vi "Sort Frames by Timing.vi"(8 "error in (no error)":errorcluster, 9 "Counter Offset":i32=3, 10 "Max frames per bucket":i32=10, 11 "Outgoing Cyclic Frames":T4[](array[typedef])=[{"Type"=enum."Periodic", "Frame ID"=101, "Payload Length"=8, "VS Offset"=0, "VS Length"=2, "Frame Conversion"="", "Frame.Data"=[0.0, 0.0], "Generation Period"=100, "Time Since Last Generation"=0, "Generation Iterations"=10, "Generation Counter"=0, "Has Protection?"=FALSE, "Protection Configurations"=[], "Has Counter?"=FALSE, "Counter Configurations"=[], "Has Disable?"=FALSE, "Disable VS Index"=0, "Transmit Trigger"=enum."Channel value change", "Trigger VS Index"=0}, {"Type"=enum."Periodic", "Frame ID"=110, "Payload Length"=8, "VS Offset"=2, "VS Length"=2, "Frame Conversion"="", "Frame.Data"=[0.0, 0.0], "Generation Period"=100, "Time Since Last Generation"=0, "Generation Iterations"=10, "Generation Counter"=0, "Has Protection?"=FALSE, "Protection Configurations"=[], "Has Counter?"=FALSE, "Counter Configurations"=[], "Has Disable?"=FALSE, "Disable VS Index"=0, "Transmit Trigger"=enum."Channel value change", "Trigger VS Index"=0}, {"Type"=enum."Periodic", "Frame ID"=1, "Payload Length"=8, "VS Offset"=4, "VS Length"=2, "Frame Conversion"="", "Frame.Data"=[0.0, 0.0], "Generation Period"=10, "Time Since Last Generation"=0, "Generation Iterations"=1, "Generation Counter"=0, "Has Protection?"=FALSE, "Protection Configurations"=[], "Has Counter?"=FALSE, "Counter Configurations"=[], "Has Disable?"=FALSE, "Disable VS Index"=0, "Transmit Trigger"=enum."Channel value change", "Trigger VS Index"=0}, {"Type"=enum."Periodic", "Frame ID"=51, "Payload Length"=8, "VS Offset"=8, "VS Length"=2, "Frame Conversion"="", "Frame.Data"=[0.0, 0.0], "Generation Period"=50, "Time Since Last Generation"=0, "Generation Iterations"=5, "Generation Counter"=0, "Has Protection?"=FALSE, "Protection Configurations"=[], "Has Counter?"=FALSE, "Counter Configurations"=[], "Has Disable?"=FALSE, "Disable VS Index"=0, "Transmit Trigger"=enum."Channel value change", "Trigger VS Index"=0}, {"Type"=enum."Periodic", "Frame ID"=60, "Payload Length"=8, "VS Offset"=10, "VS Length"=2, "Frame Conversion"="", "Frame.Data"=[0.0, 0.0], "Generation Period"=50, "Time Since Last Generation"=0, "Generation Iterations"=5, "Generation Counter"=0, "Has Protection?"=FALSE, "Protection Configurations"=[], "Has Counter?"=FALSE, "Counter Configurations"=[], "Has Disable?"=FALSE, "Disable VS Index"=0, "Transmit Trigger"=enum."Channel value change", "Trigger VS Index"=0}, {"Type"=enum."Periodic", "Frame ID"=102, "Payload Length"=8, "VS Offset"=12, "VS Length"=2, "Frame Conversion"="", "Frame.Data"=[0.0, 0.0], "Generation Period"=100, "Time Since Last Generation"=0, "Generation Iterations"=1, "Generation Counter"=0, "Has Protection?"=FALSE, "Protection Configurations"=[], "Has Counter?"=FALSE, "Counter Configurations"=[], "Has Disable?"=FALSE, "Disable VS Index"=0, "Transmit Trigger"=enum."Channel value change", "Trigger VS Index"=0}, {"Type"=enum."Periodic", "Frame ID"=2, "Payload Length"=8, "VS Offset"=14, "VS Length"=2, "Frame Conversion"="", "Frame.Data"=[0.0, 0.0], "Generation Period"=10, "Time Since Last Generation"=0, "Generation Iterations"=10, "Generation Counter"=0, "Has Protection?"=FALSE, "Protection Configurations"=[], "Has Counter?"=FALSE, "Counter Configurations"=[], "Has Disable?"=FALSE, "Disable VS Index"=0, "Transmit Trigger"=enum."Channel value change", "Trigger VS Index"=0}, {"Type"=enum."Periodic", "Frame ID"=52, "Payload Length"=8, "VS Offset"=16, "VS Length"=2, "Frame Conversion"="", "Frame.Data"=[], "Generation Period"=50, "Time Since Last Generation"=0, "Generation Iterations"=5, "Generation Counter"=0, "Has Protection?"=FALSE, "Protection Configurations"=[], "Has Counter?"=FALSE, "Counter Configurations"=[], "Has Disable?"=FALSE, "Disable VS Index"=0, "Transmit Trigger"=enum."Channel value change", "Trigger VS Index"=0}] {"Protection Configurations"."CRC Channels"."Data Type" items=["Signed", "Unsigned", "IEEE Float"]}) -> (0 "error out":errorcluster, 2 "Bucket of Indices":T1[](array[typedef]), 3 "Buckets of frames":T2[](array[typedef]))   [LabVIEW 2023, in "Protection and Counter Addon Engine.lvlib"]
uses:
  Protection and Counter Addon Engine.lvlib
  SubModules/Frame-Protection-Support/Source/Shared/Types/Exported Event Trigger Type.ctl
  SubModules/Frame-Protection-Support/Source/Shared/Protection and Counter Support Shared.lvlib
  SubModules/Frame-Protection-Support/Source/Shared/Types/Exported Counter Settings.ctl
  SubModules/Frame-Protection-Support/Source/Shared/Types/XNET Signal Configuration.ctl
  SubModules/Frame-Protection-Support/Source/Shared/Types/Protection Type.ctl
  SubModules/Frame-Protection-Support/Source/Engine/Types/RT Protection Configuration.ctl
  SubModules/Frame-Protection-Support/Source/Engine/Protection and Counter Support Engine.lvlib
  SubModules/Frame-Protection-Support/Source/Shared/Types/Exported Frame Type.ctl
  SubModules/Frame-Protection-Support/Source/Engine/Types/RT Frame Settings.ctl
  Types/RT Frame Settings with Index.ctl
  Types/RT Bucket of Frames.ctl
  Types/RT Bucket of Indices.ctl
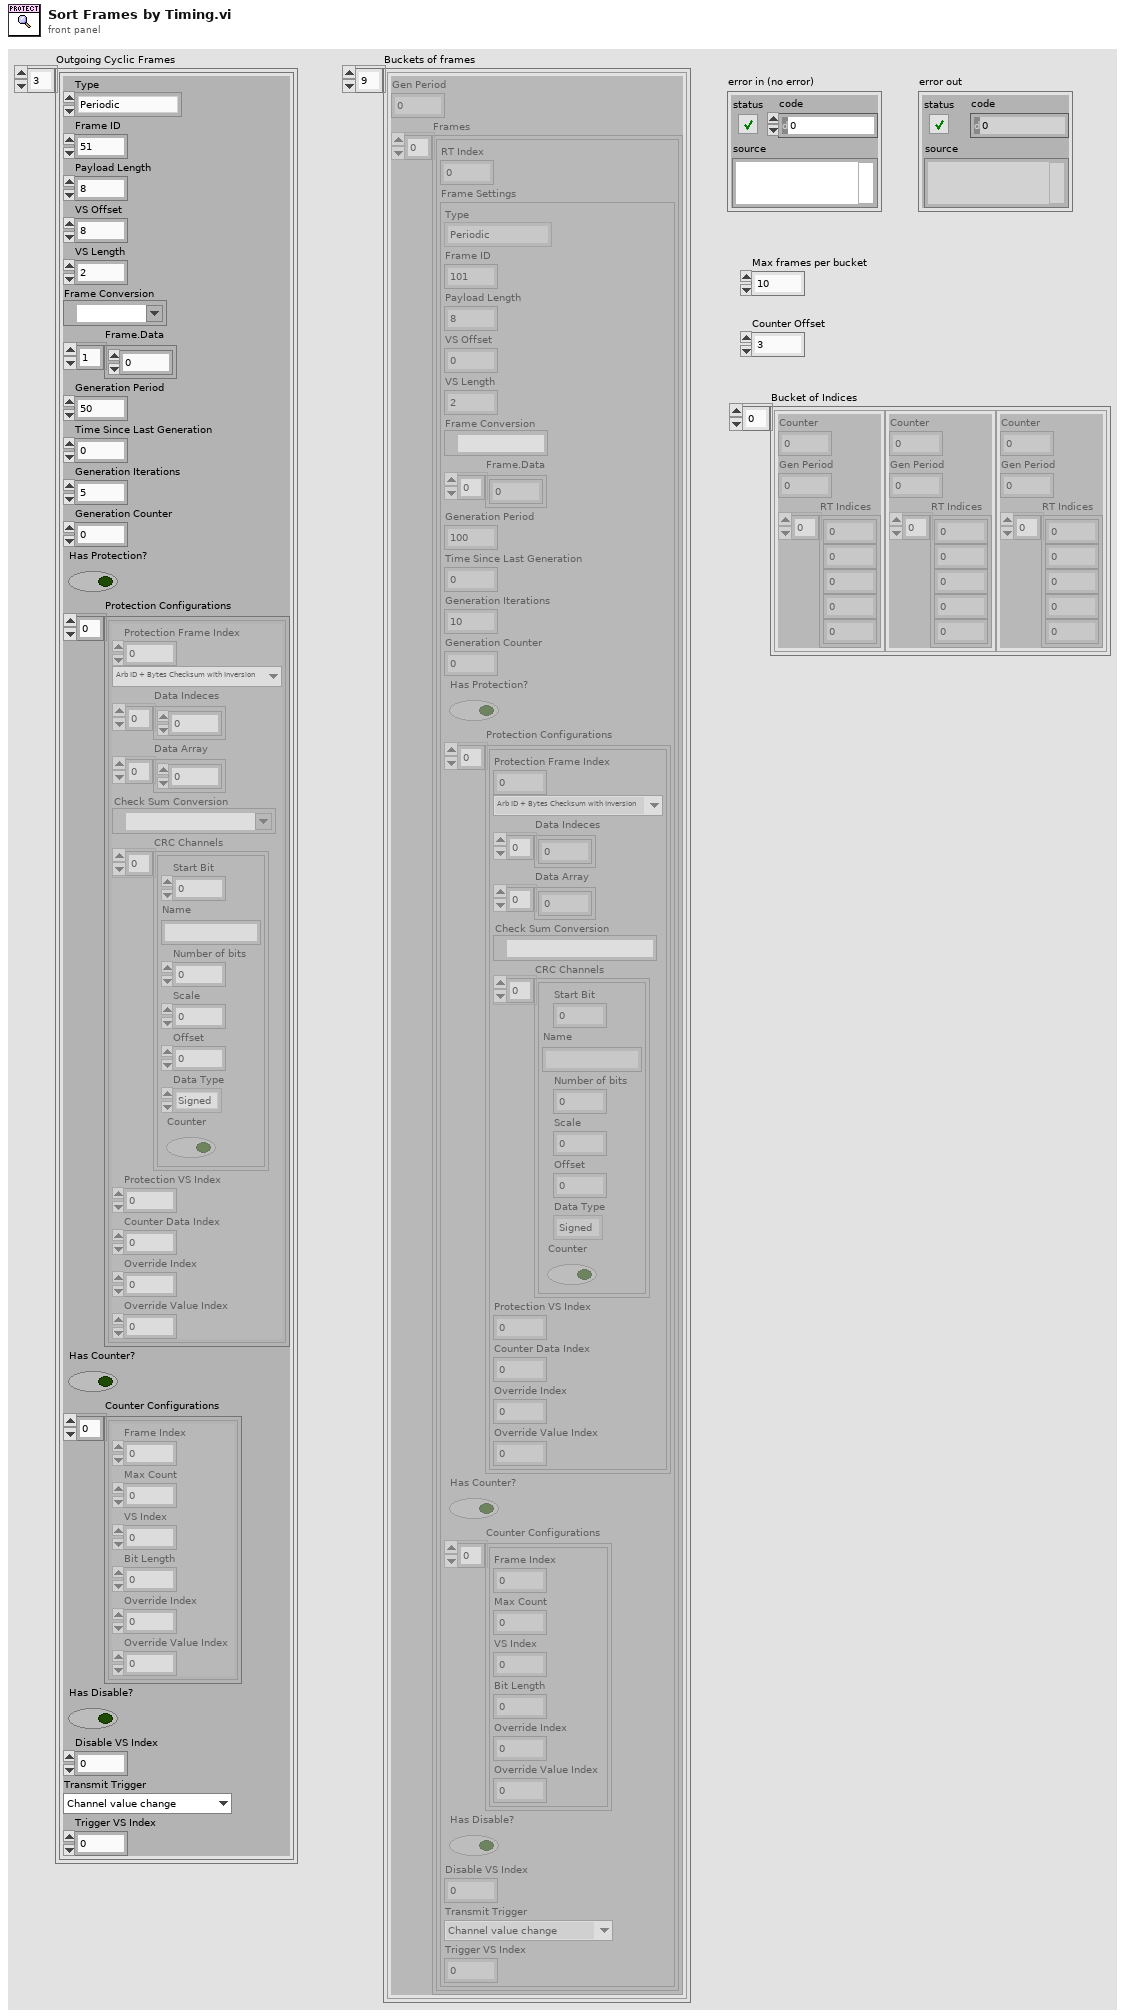
[diagram p1: front panel]
types:
  T1 = typedef "Protection and Counter Addon Engine.lvlib/RT Bucket of Indices.ctl" = cluster{"Counter":u32, "Gen Period":u32, "RT Indices":i32[]}
  T2 = typedef "Protection and Counter Addon Engine.lvlib/RT Bucket of Frames.ctl" = cluster{"Gen Period":u32, "Frames":T3[]}
  T3 = typedef "Protection and Counter Addon Engine.lvlib/RT Frame Settings with Index.ctl" = cluster{"RT Index":i32, "Frame Settings":T4}
  T4 = typedef "Protection and Counter Support Engine.lvlib/RT Frame Settings.ctl" = cluster{"Type":T5, "Frame ID":u32, "Payload Length":u32, "VS Offset":i32, "VS Length":i32, "Frame Conversion":refnum<k21>, "Frame.Data":dbl[], "Generation Period":u32, "Time Since Last Generation":u32, "Generation Iterations":u32, "Generation Counter":u32, "Has Protection?":bool, "Protection Configurations":T6[], "Has Counter?":bool, "Counter Configurations":T9[], "Has Disable?":bool, "Disable VS Index":i32, "Transmit Trigger":T10, "Trigger VS Index":i32}
  T5 = typedef "Protection and Counter Support Shared.lvlib/Exported Frame Type.ctl" = enum16{"Periodic", "Event", "Periodic/Event"}
  T6 = typedef "Protection and Counter Support Engine.lvlib/RT Protection Configuration.ctl" = cluster{"Protection Frame Index":i32, "Protection Type":T7, "Data Indeces":i32[], "Data Array":dbl[], "Check Sum Conversion":refnum<k21>, "CRC Channels":T8[], "Protection VS Index":i32, "Counter Data Index":i32, "Override Index":i32, "Override Value Index":i32}
  T7 = typedef "Protection and Counter Support Shared.lvlib/Protection Type.ctl" = enum16{"Arb ID + Bytes Checksum with Inversion", "Arb ID + Bytes CRC with Inversion", "Reversed Raw Signal Checksum with Inversion", "Concatenated Two's Compliment"}
  T8 = typedef "Protection and Counter Support Shared.lvlib/XNET Signal Configuration.ctl" = cluster{"Start Bit":i32, "Name":string, "Number of bits":i32, "Scale":dbl, "Offset":dbl, "Data Type":u32, "Counter":bool}
  T9 = typedef "Protection and Counter Support Shared.lvlib/Exported Counter Settings.ctl" = cluster{"Frame Index":i32, "Max Count":dbl, "VS Index":i32, "Bit Length":i64, "Override Index":i32, "Override Value Index":i32}
  T10 = typedef "Protection and Counter Support Shared.lvlib/Exported Event Trigger Type.ctl" = enum16{"Channel value change", "Trigger channel (not zero)", "Channel value change or trigger channel (not zero)", "Trigger channel (any value change)", "Channel value change or trigger channel (any value change)"}
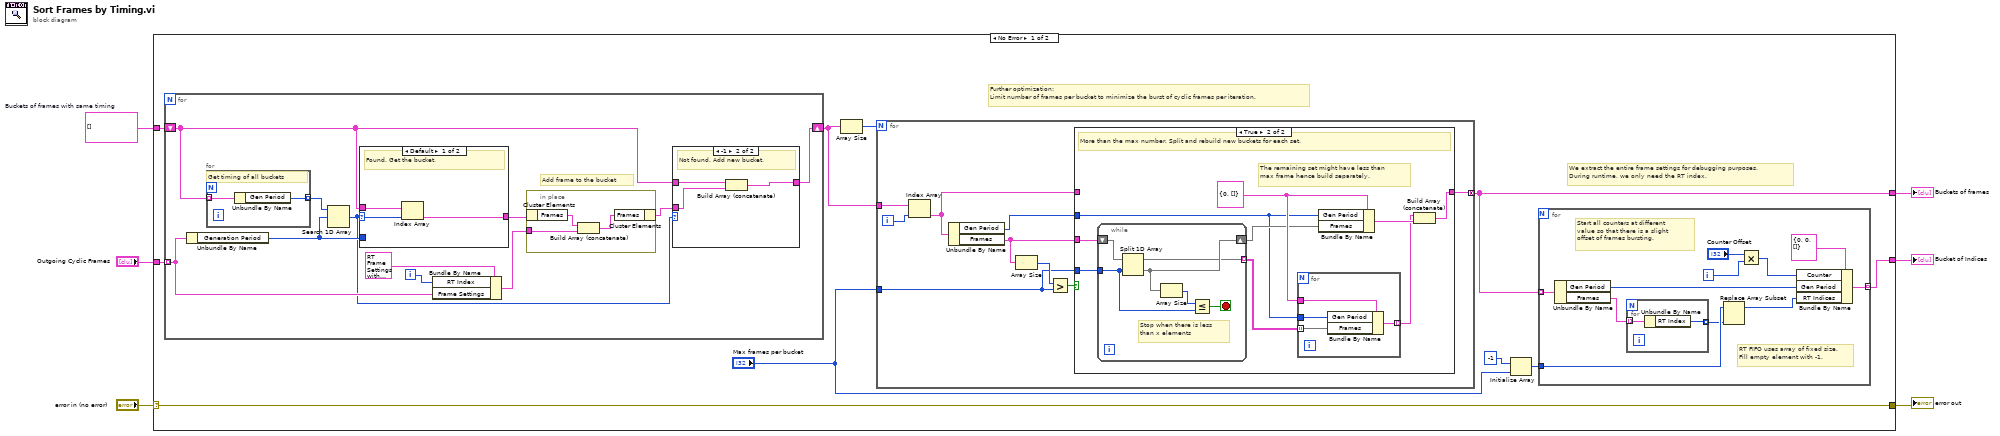
[diagram p0: block diagram]
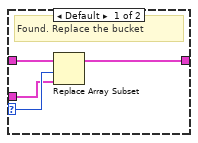
[diagram p2: hidden frame]
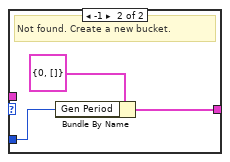
[diagram p3: hidden frame]
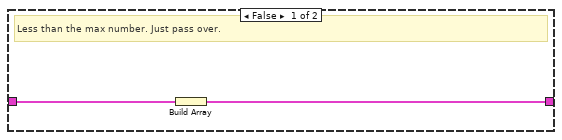
[diagram p4: hidden frame]
diagram:
  w5 = T2[] []  # Buckets of frames with same timing
  n1 = case shown="No Error" "error in (no error)" {
    selector: "error in (no error)" -> [w13 w89]
    tunnel: "Outgoing Cyclic Frames" -> [w16 _]
    tunnel: w5 -> [w15 _]
    tunnel: [w14 _] -> w2
    tunnel: [w13 w89] -> w3
    tunnel: [w10 _] -> w1
    frame No Error {
      # "We extract the entire frame settings for debugging purposes.\nDuring runtime, we only need the RT index."
      # "Further optimization:\nLimit number of frames per bucket to minimize the burst of cyclic frames per iteration."
      n2 = for {
        tunnel: w16 -> [w36] mode=indexing
        shift-right: [w30] -> w11
        shift-left: w15 -> [w31]
        i -> [w37]
        # "Add frame to the bucket"
        n3 = Unbundle By Name(w36) -> ("Generation Period"=w39:u32)
        n4 = for {
          tunnel: w31 -> [w58] mode=indexing
          tunnel: [w57] -> w40 mode=indexing
          # "Get timing of all buckets"
          n5 = Unbundle By Name(w58) -> ("Gen Period"=w57:u32)
        }
        n6 = Search 1D Array(1D array=w40, element=w39) -> (index of element=w32:i32)  [unwired: 1 in]
        n7 = case shown="Default" w32 {
          selector: w32 -> [w52 _]
          tunnel: w39 -> [_ w55]
          tunnel: w31 -> [w53 _]
          tunnel: [w51 w54] -> w35
          frame Default {
            # "Found. Get the bucket."
            n8 = Index Array(array=w53, index=w52) -> (element=w51:T2)
          }
          frame -1 {
            # "Not found. Create a new bucket."
            n9 = Bundle By Name(cluster=T2 {"Gen Period"=0, "Frames"=[]}, "Gen Period"=w55) -> (w54:T2)
          }
        }
        n10 = Bundle By Name(cluster=T3 {"RT Index"=0, "Frame Settings"={"Type"=enum."Periodic", "Frame ID"=101, "Payload Length"=8, "VS Offset"=0, "VS Length"=2, "Frame Conversion"="", "Frame.Data"=[0.0, 0.0], "Generation Period"=100, "Time Since Last Generation"=0, "Generation Iterations"=10, "Generation Counter"=0, "Has Protection?"=FALSE, "Protection Configurations"=[], "Has Counter?"=FALSE, "Counter Configurations"=[], "Has Disable?"=FALSE, "Disable VS Index"=0, "Transmit Trigger"=enum."Channel value change", "Trigger VS Index"=0}}, "RT Index"=w37, "Frame Settings"=w36) -> (w34:T3)
        n11 = in-place {
          in-place-border: w34 -> [w48]
          n12 = in-place-cluster #1(w35) -> ("Frames"=w49:T3[])
          n13 = Build Array (concatenate)(w49, w48) -> (w50:T3[])
          n14 = in-place-cluster #1("Frames"=w50) -> (w33:T2)
        }
        n15 = case shown="-1" w32 {
          selector: w32 -> [w43 _]
          tunnel: w33 -> [w42 w46]
          tunnel: w31 -> [w44 w47]
          tunnel: [w41 w45] -> w30
          frame Default {
            # "Found. Replace the bucket"
            n16 = Replace Array Subset(array=w44, new element=w42, index=w43) -> (w41:T2[])
          }
          frame -1 {
            # "Not found. Add new bucket."
            n17 = Build Array (concatenate)(w47, w46) -> (w45:T2[])
          }
        }
      }
      n18 = Array Size(array=w11) -> (size(s)=w12:i32)
      n19 = for {
        N: w12 -> [_]
        tunnel: "Max frames per bucket" -> [w64]
        tunnel: [w62] -> w14 mode=concatenating
        tunnel: w11 -> [w61]
        i -> [w60]
        n20 = Index Array(array=w61, index=w60) -> (element=w59:T2)
        n21 = Unbundle By Name(w59) -> ("Gen Period"=w63:u32, "Frames"=w65:T3[])
        n22 = Array Size(array=w65) -> (size(s)=w67:i32)
        n23 = Greater?(x=w67, y=w64) -> (0:w66:bool)
        n24 = case shown="True" w66 {
          tunnel: w65 -> [_ w78]
          tunnel: w64 -> [_ w77]
          tunnel: w63 -> [_ w73]
          tunnel: w59 -> [w69 _]
          tunnel: [w68 w70] -> w62
          frame False {
            # "Less than the max number. Just pass over."
            n25 = Build Array(w69) -> (w68:T2[])
          }
          frame True {
            w75 = T2 {"Gen Period"=0, "Frames"=[]}
            # "The remaining set might have less than max frame hence build separately."
            # "More than the max number. Split and rebuild new buckets for each set."
            n26 = while {
              tunnel: w77 -> [w81]
              shift-right: [w83] -> w74
              shift-left: w78 -> [w84]
              tunnel: [w79] -> w76 mode=indexing
              stop <- w80 stop-if-true
              # "Stop when there is less than x elements"
              n27 = Split 1D Array(array=w84, index=w81) -> (first subarray=w79:T3[], second subarray=w83:T3[])
              n28 = Array Size(array=w83) -> (size(s)=w82:i32)
              n29 = Less Or Equal?(x=w82, y=w81) -> (x <= y?=w80:bool)
            }
            n30 = for {
              tunnel: w73 -> [w88]
              tunnel: w75 -> [w87]
              tunnel: w76 -> [w86] mode=indexing
              tunnel: [w85] -> w71 mode=indexing
              n31 = Bundle By Name(cluster=w87, "Gen Period"=w88, "Frames"=w86) -> (w85:T2)
            }
            n32 = Bundle By Name(cluster=w75, "Gen Period"=w73, "Frames"=w74) -> (w72:T2)
            n33 = Build Array (concatenate)(w71, w72) -> (w70:T2[])
          }
        }
      }
      n34 = Initialize Array(-1 ("RT Index"), "Max frames per bucket") -> (w7:i32[])
      n35 = for {
        tunnel: w14 -> [w27] mode=indexing
        tunnel: [w24] -> w10 mode=indexing
        tunnel: w7 -> [w23]
        i -> [w20]
        # "RT FIFO uses array of fixed size.\nFill empty element with -1."
        # "Start all counters at different value so that there is a slight offset of frames bursting."
        n36 = Unbundle By Name(w27) -> ("Gen Period"=w17:u32, "Frames"=w26:T3[])
        n37 = for {
          tunnel: w26 -> [w29] mode=indexing
          tunnel: [w28] -> w22 mode=indexing
          n38 = Unbundle By Name(w29) -> ("RT Index"=w28:i32)
        }
        n39 = Replace Array Subset(array=w23, new element=w22) -> (w21:i32[])  [unwired: 1 in]
        n40 = Multiply(x="Counter Offset", y=w20) -> (x*y=w18:i32)
        n41 = Bundle By Name(cluster=T1 {"Counter"=0, "Gen Period"=0, "RT Indices"=[]} ("Bucket of Frames"), "Counter"=w18, "Gen Period"=w17, "RT Indices"=w21) -> (w24:T1)
      }
    }
    frame Error {
    }
  }
  "error out" <- w3
  "Buckets of frames" <- w2
  "Bucket of Indices" <- w1
